vi "output.vi"(8 "error in":errorcluster, 10 "data table in":T1, 11 "SystemLin Tag Module runtime in":refnum<class "SystemLink runtime.lvclass">) -> (0 "error out":errorcluster, 2 "data table out":T1, 3 "SystemLin Tag Module runtime out":refnum<class "SystemLink runtime.lvclass">)   [LabVIEW 2015, in "SystemLink runtime.lvclass"]
doc: "Provides an interface for writing data to a module at runtime. While this interface performs no operations, a child should provide an override which may write to any open sessions, references, or interfaces."
uses:
  SystemLink runtime.lvclass
  <vilib>/NI/Tag Bus/table/data table.ctl
  SystemLink runtime.lvclass/SystemLink runtime.ctl
  <vilib>/NI/Tag Bus/table/data polymorphs/read one/read Double.vi
  <vilib>/NI/Tag Bus/table/data polymorphs/read one/read U64.vi
  <vilib>/NI/Tag Bus/table/data polymorphs/read one/read U32.vi
  <vilib>/NI/Tag Bus/table/data polymorphs/read one/read U16.vi
  <vilib>/NI/Tag Bus/table/data polymorphs/read one/read U8.vi
  <vilib>/NI/Tag Bus/table/data polymorphs/read one/read Single.vi
  <vilib>/NI/Tag Bus/table/data polymorphs/read one/read I32.vi
  <vilib>/NI/Tag Bus/table/data polymorphs/read one/read I16.vi
  <vilib>/NI/Tag Bus/table/data polymorphs/read one/read I8.vi
  <vilib>/NI/Tag Bus/table/data polymorphs/read one/read Boolean.vi
  <vilib>/NI/Tag Bus/table/data polymorphs/read one/read String.vi
  <vilib>/NI/Tag Bus/table/data table.lvlib
  <vilib>/Skyline/Tag/Wrapper/Wrapper_class/NI Skyline Tag.lvclass
  <vilib>/Skyline/Tag/Wrapper/Wrapper_class/Write Tag (DBL).vi
  <vilib>/Skyline/Tag/Wrapper/Wrapper_class/Write Tag (I32).vi
  <vilib>/Skyline/Tag/Wrapper/Wrapper_class/Write Tag (String).vi
  <vilib>/Skyline/Tag/Wrapper/Wrapper AMQP_class/NI Skyline Tag AMQP.lvclass
  <vilib>/Skyline/Tag/Shared/NI Skyline Tag.lvlib
  <vilib>/Skyline/Tag/Wrapper/Wrapper HTTP_class/NI Skyline Tag HTTP.lvclass
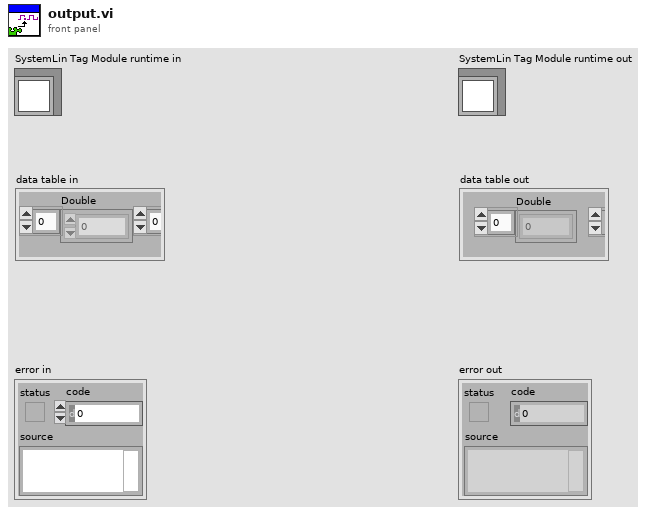
[diagram p1: front panel]
types:
  T1 = typedef "tag bus.lvlib/data table.lvlib/data table.ctl" = cluster{"Double":dbl[], "Single":sgl[], "I64":i64[], "I32":i32[], "I16":i16[], "I8":i8[], "U64":u64[], "U32":u32[], "U16":u16[], "U8":u8[], "Boolean":bool[], "String":string[], "Array of Double":cluster{"DBL Array":dbl[]}[], "Array of Single":cluster{"SGL Array":sgl[]}[], "Array of I64":cluster{"I64 Array":i64[]}[], "Array of I32":cluster{"I32 Array":i32[]}[], "Array of I16":cluster{"I16 Array":i16[]}[], "Array of I8":cluster{"I8 Array":i8[]}[], "Array of U64":cluster{"U64 Array":u64[]}[], "Array of U32":cluster{"U32 Array":u32[]}[], "Array of U16":cluster{"U16 Array":u16[]}[], "Array of U8":cluster{"U8 Array":u8[]}[], "Array of Boolean":cluster{"Boolean Array":bool[]}[], "Array of String":cluster{"String Array":string[]}[]}
  T2 = typedef "SystemLink configuration.lvclass/SysLink Mapping.ctl" = cluster{"Data Type":T3, "Tag Reference":refnum<class "NI Skyline Tag.lvclass">, "Tag Bus Index":i32, "AMQP":bool, "Skylink Index":i32}
  T3 = typedef "SystemLink configuration.lvclass/Data Tag Type.ctl" = enum16{"Double", "Single", "I32", "I16", "I8", "U64", "U32", "U16", "U8", "Boolean", "String", "Timestamp"}
  T4 = typedef "NI Skyline Tag.lvclass/Tag Value Cluster Wrapper.ctl" = cluster{"Configuration":refnum<class "NI Skyline Configuration.lvclass">, "Tag Cluster":T5}
  T5 = typedef "NI Skyline Tag.lvlib/Tag Value Cluster.ctl" = cluster{"Path":string, "Data Type":T6, "Value":string, "Time Stamp":timestamp}
  T6 = typedef "NI Skyline Tag.lvlib/DataType.ctl" = enum32{"Double", "I32", "String", "Boolean", "U64", "Timestamp"}
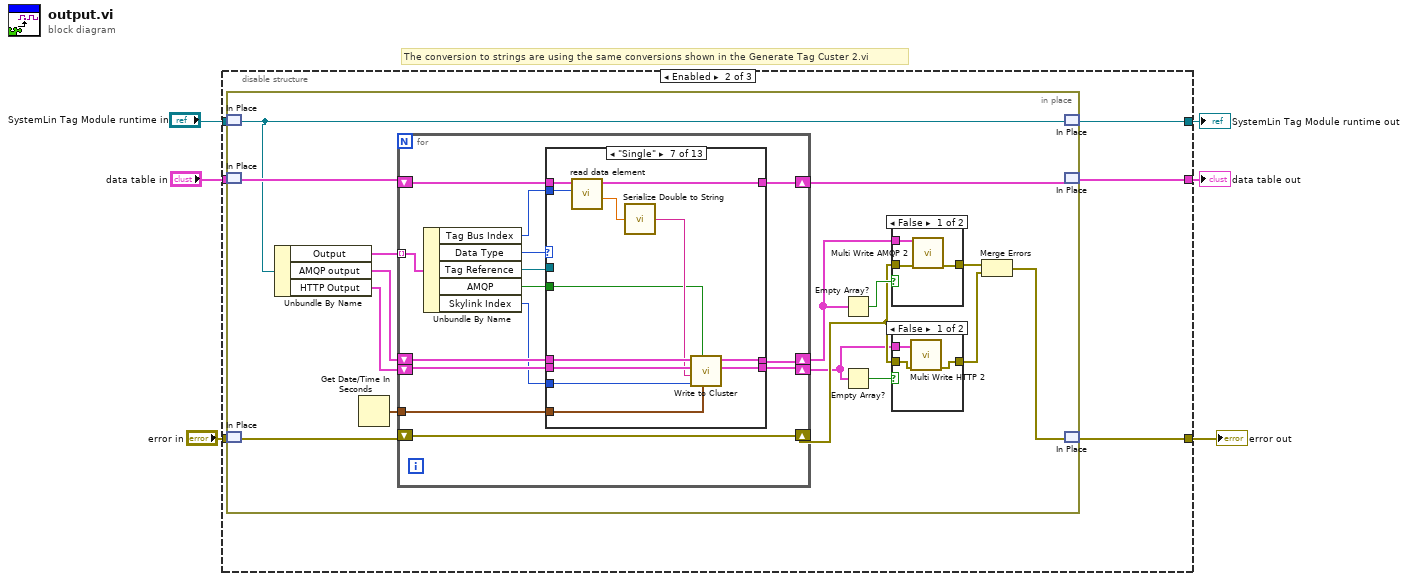
[diagram p0: block diagram]
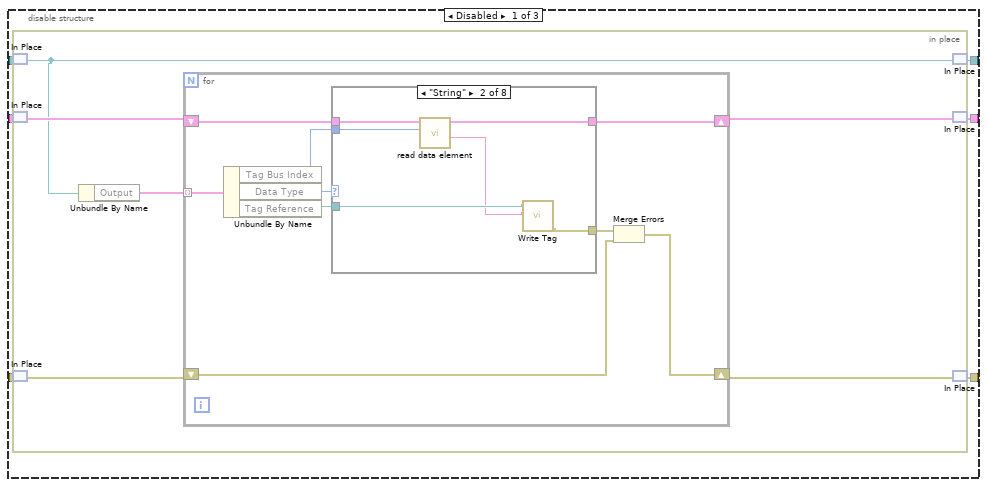
[diagram p2: hidden frame]
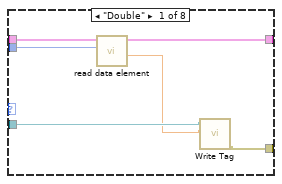
[diagram p3: hidden frame]
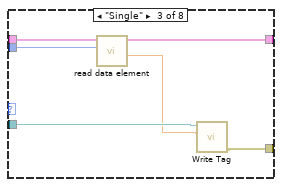
[diagram p4: hidden frame]
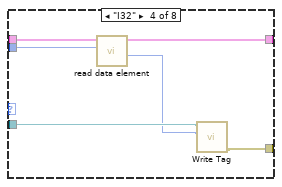
[diagram p5: hidden frame]
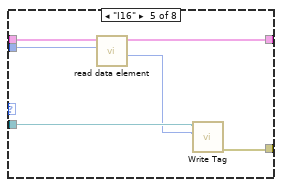
[diagram p6: hidden frame]
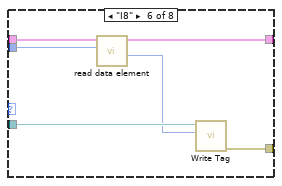
[diagram p7: hidden frame]
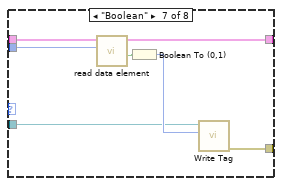
[diagram p8: hidden frame]
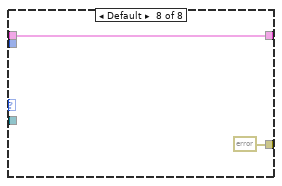
[diagram p9: hidden frame]
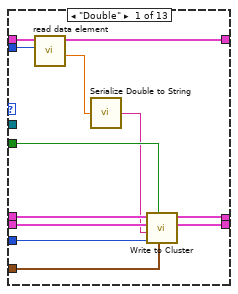
[diagram p12: hidden frame]
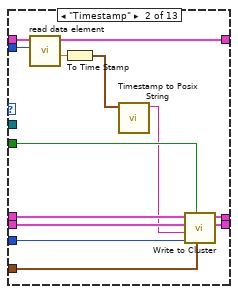
[diagram p13: hidden frame]
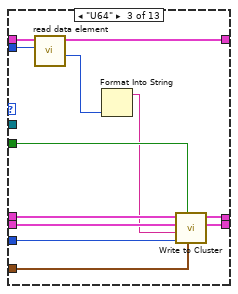
[diagram p14: hidden frame]
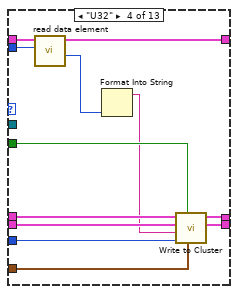
[diagram p15: hidden frame]
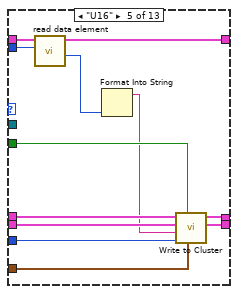
[diagram p16: hidden frame]
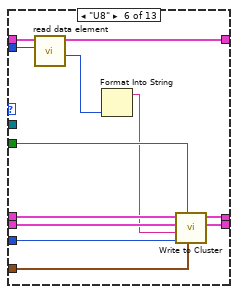
[diagram p17: hidden frame]
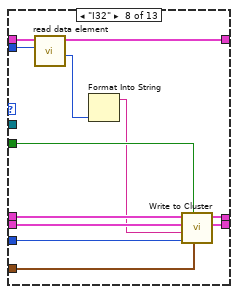
[diagram p18: hidden frame]
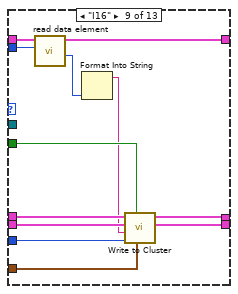
[diagram p19: hidden frame]
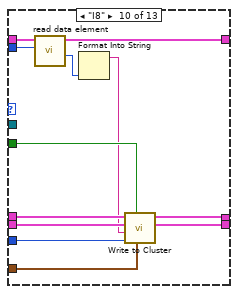
[diagram p20: hidden frame]
diagram:
  # "The conversion to strings are using the same conversions shown in the Generate Tag Custer 2.vi"
  n1 = disable-structure shown="Enabled" {
    disable-tunnel: "SystemLin Tag Module runtime in" -> [w12 w78 _]
    disable-tunnel: [w11 w77 _] -> w5
    disable-tunnel: [w10 w76 _] -> w4
    disable-tunnel: [w9 w75 _] -> w3
    disable-tunnel: "data table in" -> [w8 w74 _]
    disable-tunnel: "error in" -> [w7 w73 _]
    frame Disabled {
      n2 = in-place {
        n3 = in-place-match #1(w12) -> (w16:refnum<class "SystemLink runtime.lvclass">)
        n4 = in-place-match #2(w8) -> (w18:T1)
        n5 = in-place-match #3(w7) -> (w14:errorcluster)
        n6 = Unbundle By Name(w16) -> ("Output"=w15:T2[])
        n7 = for {
          shift-right: [w24] -> w17
          shift-left: w18 -> [w25]
          tunnel: w15 -> [w27] mode=indexing
          shift-right: [w19] -> w13
          shift-left: w14 -> [w20]
          n8 = Unbundle By Name(w27) -> ("Tag Bus Index"=w22:i32, "Data Type"=w26:T3, "Tag Reference"=w23:refnum<class "NI Skyline Tag.lvclass">)
          n9 = case shown="\"String\"" w26 {
            tunnel: w25 -> [w33 w39 w45 w51 w57 w63 w70 w72]
            tunnel: [w31 w37 w43 w49 w55 w61 w68 w72] -> w24
            tunnel: w23 -> [w30 w36 w42 w48 w54 w60 w64 _]
            tunnel: [w28 w34 w40 w46 w52 w58 w67 errorcluster {"status"=FALSE, "code"=0, "source"=""} ("error IO")] -> w21
            tunnel: w22 -> [w32 w38 w44 w50 w56 w62 w69 _]
            frame "Double" {
              n10 = call-poly <vilib>:"read data element.vi"("index"=w32, "data table in"=w33) -> ("value"=w29:dbl, "data table out"=w31:T1)  [unwired: 8 in]
              n11 = call-poly <vilib>:"Write Tag.vi"("value"=w29, "tag in"=w30) -> ("error out"=w28:errorcluster)  [unwired: 8 in, 1 out]
            }
            frame "String" {
              n12 = call-poly <vilib>:"read data element.vi"("index"=w38, "data table in"=w39) -> ("value"=w35:string, "data table out"=w37:T1)  [unwired: 8 in]
              n13 = call-poly <vilib>:"Write Tag.vi"("value"=w35, "tag in"=w36) -> ("error out"=w34:errorcluster)  [unwired: 8 in, 1 out]
            }
            frame "Single" {
              n14 = call-poly <vilib>:"read data element.vi"("index"=w44, "data table in"=w45) -> ("value"=w41:sgl, "data table out"=w43:T1)  [unwired: 8 in]
              n15 = call-poly <vilib>:"Write Tag.vi"("value"=w41, "tag in"=w42) -> ("error out"=w40:errorcluster)  [unwired: 8 in, 1 out]
            }
            frame "I32" {
              n16 = call-poly <vilib>:"read data element.vi"("index"=w50, "data table in"=w51) -> ("value"=w47:i32, "data table out"=w49:T1)  [unwired: 8 in]
              n17 = call-poly <vilib>:"Write Tag.vi"("value"=w47, "tag in"=w48) -> ("error out"=w46:errorcluster)  [unwired: 8 in, 1 out]
            }
            frame "I16" {
              n18 = call-poly <vilib>:"read data element.vi"("index"=w56, "data table in"=w57) -> ("value"=w53:i16, "data table out"=w55:T1)  [unwired: 8 in]
              n19 = call-poly <vilib>:"Write Tag.vi"("value"=w53, "tag in"=w54) -> ("error out"=w52:errorcluster)  [unwired: 8 in, 1 out]
            }
            frame "I8" {
              n20 = call-poly <vilib>:"read data element.vi"("index"=w62, "data table in"=w63) -> ("value"=w59:i8, "data table out"=w61:T1)  [unwired: 8 in]
              n21 = call-poly <vilib>:"Write Tag.vi"("value"=w59, "tag in"=w60) -> ("error out"=w58:errorcluster)  [unwired: 8 in, 1 out]
            }
            frame "Boolean" {
              n22 = call-poly <vilib>:"read data element.vi"("index"=w69, "data table in"=w70) -> ("value"=w65:bool, "data table out"=w68:T1)  [unwired: 8 in]
              n23 = Boolean To (0,1)(Boolean=w65) -> (0, 1=w66:i16)
              n24 = call-poly <vilib>:"Write Tag.vi"("value"=w66, "tag in"=w64) -> ("error out"=w67:errorcluster)  [unwired: 8 in, 1 out]
            }
            frame Default {
            }
          }
          n25 = Merge Errors(w21, w20) -> (w19:errorcluster)
        }
        n26 = in-place-match #1(w16) -> (w11:refnum<class "SystemLink runtime.lvclass">)
        n27 = in-place-match #2(w17) -> (w10:T1)
        n28 = in-place-match #3(w13) -> (w9:errorcluster)
      }
    }
    frame Enabled {
      n29 = in-place {
        n30 = in-place-match #4(w78) -> (w92:refnum<class "SystemLink runtime.lvclass">)
        n31 = in-place-match #5(w74) -> (w94:T1)
        n32 = in-place-match #6(w73) -> (w90:errorcluster)
        n33 = Unbundle By Name(w92) -> ("Output"=w91:T2[], "AMQP output"=w89:T4[], "HTTP Output"=w88:T4[])
        n34 = Get Date/Time In Seconds() -> (seconds since 1Jan1904=w79:timestamp)
        n35 = for {
          shift-right: [w113] -> w93
          shift-left: w94 -> [w114]
          tunnel: w91 -> [w116] mode=indexing
          shift-right: [w110] -> w83
          shift-left: w90 -> [w110]
          shift-right: [w104] -> w81
          shift-left: w88 -> [w108]
          shift-right: [w105] -> w80
          shift-left: w89 -> [w109]
          tunnel: w79 -> [w103]
          n36 = Unbundle By Name(w116) -> ("Tag Bus Index"=w111:i32, "Data Type"=w115:T3, "Tag Reference"=w112:refnum<class "NI Skyline Tag.lvclass">, "AMQP"=w107:bool, "Skylink Index"=w106:i32)
          n37 = case shown="\"Single\"" w115 {
            tunnel: w114 -> [w128 w141 w153 w165 w177 w189 w201 w213 w225 w237 w251 w262 w265]
            tunnel: [w126 w139 w151 w163 w175 w187 w199 w211 w223 w235 w249 w260 w265] -> w113
            tunnel: w112 -> [_ _ _ _ _ _ _ _ _ _ _ _ _]
            tunnel: w111 -> [w127 w140 w152 w164 w176 w188 w200 w212 w224 w236 w250 w261 _]
            tunnel: w109 -> [w125 w138 w150 w162 w174 w186 w198 w210 w222 w234 w248 w257 w264]
            tunnel: w108 -> [w124 w137 w149 w161 w173 w185 w197 w209 w221 w233 w247 w256 w263]
            tunnel: w107 -> [w119 w132 w144 w156 w168 w180 w190 w204 w216 w228 w242 w255 _]
            tunnel: w106 -> [w120 w133 w145 w157 w169 w181 w193 w205 w217 w229 w243 w253 _]
            tunnel: [w123 w136 w148 w160 w172 w184 w196 w208 w220 w232 w246 w259 w264] -> w105
            tunnel: [w122 w135 w147 w159 w171 w183 w195 w207 w219 w231 w245 w258 w263] -> w104
            tunnel: w103 -> [w121 w134 w146 w158 w170 w182 w194 w206 w218 w230 w244 w254 _]
            frame "Double" {
              n38 = call-poly <vilib>:"read data element.vi"("index"=w127, "data table in"=w128) -> ("value"=w118:dbl, "data table out"=w126:T1)  [unwired: 8 in]
              n39 = call <vilib>:"Serialize Double to String.vi"("double"=w118) -> ("string"=w117:string)
              n40 = call "Write to Cluster.vi"("Tag Cluster.Time Stamp"=w121, "AMQP"=w119, "Skylink Index"=w120, "String"=w117, "HTTP  in"=w124, "AMQP  in"=w125) -> ("HTTP  out"=w122:T4[], "AMQP  out"=w123:T4[])  [unwired: 4 in]
            }
            frame "Timestamp" {
              n41 = call-poly <vilib>:"read data element.vi"("index"=w140, "data table in"=w141) -> ("value"=w131:dbl, "data table out"=w139:T1)  [unwired: 8 in]
              n42 = To Time Stamp(1:w131) -> (0:w130:timestamp)
              n43 = call <vilib>:"Timestamp to Posix String.vi"("time stamp"=w130) -> ("posix time string"=w129:string)  [unwired: 10 in]
              n44 = call "Write to Cluster.vi"("Tag Cluster.Time Stamp"=w134, "AMQP"=w132, "Skylink Index"=w133, "String"=w129, "HTTP  in"=w137, "AMQP  in"=w138) -> ("HTTP  out"=w135:T4[], "AMQP  out"=w136:T4[])  [unwired: 4 in]
            }
            frame "U64" {
              n45 = call-poly <vilib>:"read data element.vi"("index"=w152, "data table in"=w153) -> ("value"=w143:u64, "data table out"=w151:T1)  [unwired: 8 in]
              n46 = Format Into String(w143) -> (resulting string=w142:string)  [unwired: 3 in, 1 out]
              n47 = call "Write to Cluster.vi"("Tag Cluster.Time Stamp"=w146, "AMQP"=w144, "Skylink Index"=w145, "String"=w142, "HTTP  in"=w149, "AMQP  in"=w150) -> ("HTTP  out"=w147:T4[], "AMQP  out"=w148:T4[])  [unwired: 4 in]
            }
            frame "U32" {
              n48 = call-poly <vilib>:"read data element.vi"("index"=w164, "data table in"=w165) -> ("value"=w155:u32, "data table out"=w163:T1)  [unwired: 8 in]
              n49 = Format Into String(w155) -> (resulting string=w154:string)  [unwired: 3 in, 1 out]
              n50 = call "Write to Cluster.vi"("Tag Cluster.Time Stamp"=w158, "AMQP"=w156, "Skylink Index"=w157, "String"=w154, "HTTP  in"=w161, "AMQP  in"=w162) -> ("HTTP  out"=w159:T4[], "AMQP  out"=w160:T4[])  [unwired: 4 in]
            }
            frame "U16" {
              n51 = call-poly <vilib>:"read data element.vi"("index"=w176, "data table in"=w177) -> ("value"=w167:u16, "data table out"=w175:T1)  [unwired: 8 in]
              n52 = Format Into String(w167) -> (resulting string=w166:string)  [unwired: 3 in, 1 out]
              n53 = call "Write to Cluster.vi"("Tag Cluster.Time Stamp"=w170, "AMQP"=w168, "Skylink Index"=w169, "String"=w166, "HTTP  in"=w173, "AMQP  in"=w174) -> ("HTTP  out"=w171:T4[], "AMQP  out"=w172:T4[])  [unwired: 4 in]
            }
            frame "U8" {
              n54 = call-poly <vilib>:"read data element.vi"("index"=w188, "data table in"=w189) -> ("value"=w179:u8, "data table out"=w187:T1)  [unwired: 8 in]
              n55 = Format Into String(w179) -> (resulting string=w178:string)  [unwired: 3 in, 1 out]
              n56 = call "Write to Cluster.vi"("Tag Cluster.Time Stamp"=w182, "AMQP"=w180, "Skylink Index"=w181, "String"=w178, "HTTP  in"=w185, "AMQP  in"=w186) -> ("HTTP  out"=w183:T4[], "AMQP  out"=w184:T4[])  [unwired: 4 in]
            }
            frame "Single" {
              n57 = call-poly <vilib>:"read data element.vi"("index"=w200, "data table in"=w201) -> ("value"=w192:sgl, "data table out"=w199:T1)  [unwired: 8 in]
              n58 = call <vilib>:"Serialize Double to String.vi"("double"=w192) -> ("string"=w191:string)
              n59 = call "Write to Cluster.vi"("Tag Cluster.Time Stamp"=w194, "AMQP"=w190, "Skylink Index"=w193, "String"=w191, "HTTP  in"=w197, "AMQP  in"=w198) -> ("HTTP  out"=w195:T4[], "AMQP  out"=w196:T4[])  [unwired: 4 in]
            }
            frame "I32" {
              n60 = call-poly <vilib>:"read data element.vi"("index"=w212, "data table in"=w213) -> ("value"=w203:i32, "data table out"=w211:T1)  [unwired: 8 in]
              n61 = Format Into String(w203) -> (resulting string=w202:string)  [unwired: 3 in, 1 out]
              n62 = call "Write to Cluster.vi"("Tag Cluster.Time Stamp"=w206, "AMQP"=w204, "Skylink Index"=w205, "String"=w202, "HTTP  in"=w209, "AMQP  in"=w210) -> ("HTTP  out"=w207:T4[], "AMQP  out"=w208:T4[])  [unwired: 4 in]
            }
            frame "I16" {
              n63 = call-poly <vilib>:"read data element.vi"("index"=w224, "data table in"=w225) -> ("value"=w215:i16, "data table out"=w223:T1)  [unwired: 8 in]
              n64 = Format Into String(w215) -> (resulting string=w214:string)  [unwired: 3 in, 1 out]
              n65 = call "Write to Cluster.vi"("Tag Cluster.Time Stamp"=w218, "AMQP"=w216, "Skylink Index"=w217, "String"=w214, "HTTP  in"=w221, "AMQP  in"=w222) -> ("HTTP  out"=w219:T4[], "AMQP  out"=w220:T4[])  [unwired: 4 in]
            }
            frame "I8" {
              n66 = call-poly <vilib>:"read data element.vi"("index"=w236, "data table in"=w237) -> ("value"=w227:i8, "data table out"=w235:T1)  [unwired: 8 in]
              n67 = Format Into String(w227) -> (resulting string=w226:string)  [unwired: 3 in, 1 out]
              n68 = call "Write to Cluster.vi"("Tag Cluster.Time Stamp"=w230, "AMQP"=w228, "Skylink Index"=w229, "String"=w226, "HTTP  in"=w233, "AMQP  in"=w234) -> ("HTTP  out"=w231:T4[], "AMQP  out"=w232:T4[])  [unwired: 4 in]
            }
            frame "Boolean" {
              n69 = call-poly <vilib>:"read data element.vi"("index"=w250, "data table in"=w251) -> ("value"=w239:bool, "data table out"=w249:T1)  [unwired: 8 in]
              n70 = Select(t="True", s=w239, f="False") -> (s? t:f=w238:string)
              n71 = call "Write to Cluster.vi"("Tag Cluster.Time Stamp"=w244, "AMQP"=w242, "Skylink Index"=w243, "String"=w238, "HTTP  in"=w247, "AMQP  in"=w248) -> ("HTTP  out"=w245:T4[], "AMQP  out"=w246:T4[])  [unwired: 4 in]
            }
            frame "String" {
              n72 = call-poly <vilib>:"read data element.vi"("index"=w261, "data table in"=w262) -> ("value"=w252:string, "data table out"=w260:T1)  [unwired: 8 in]
              n73 = call "Write to Cluster.vi"("Tag Cluster.Time Stamp"=w254, "AMQP"=w255, "Skylink Index"=w253, "String"=w252, "HTTP  in"=w256, "AMQP  in"=w257) -> ("HTTP  out"=w258:T4[], "AMQP  out"=w259:T4[])  [unwired: 4 in]
            }
            frame Default {
              (unwired) errorcluster {"status"=FALSE, "code"=0, "source"=""} ("error IO")
            }
          }
        }
        n74 = Empty Array?(array=w80) -> (empty?=w86:bool)
        n75 = Empty Array?(array=w81) -> (empty?=w87:bool)
        n76 = case shown="False" w86 {
          tunnel: [w99 w102] -> w85
          tunnel: w80 -> [w101 _]
          tunnel: w83 -> [w100 w102]
          frame False {
            n77 = call <vilib>:"Multi Write AMQP 2.vi"("error in (no error)"=w100, "tags in"=w101) -> ("error out"=w99:errorcluster)  [unwired: 9 in]
          }
          frame True {
          }
        }
        n78 = case shown="False" w87 {
          tunnel: [w95 w98] -> w84
          tunnel: w81 -> [w97 _]
          tunnel: w83 -> [w96 w98]
          frame False {
            n79 = call <vilib>:"Multi Write HTTP 2.vi"("error in (no error)"=w96, "tag clusters"=w97) -> ("error out"=w95:errorcluster)  [unwired: 9 in]
          }
          frame True {
          }
        }
        n80 = Merge Errors(w85, w84) -> (w82:errorcluster)
        n81 = in-place-match #4(w92) -> (w77:refnum<class "SystemLink runtime.lvclass">)
        n82 = in-place-match #5(w93) -> (w76:T1)
        n83 = in-place-match #6(w82) -> (w75:errorcluster)
      }
    }
    frame Disabled {
    }
  }
  "error out" <- w3
  "SystemLin Tag Module runtime out" <- w5
  "data table out" <- w4
